vi "RemoteVI Logical Popups.vi"(0 "modal popups":T2(array[cluster]), 5 "d":cluster{"dx":i32, "dy":i32}) -> (4 "popups":T1)   [LabVIEW 2020, in "RemoteVI.lvlib"]
doc: "Builds the popups cluster that RemoteVI Service Client.vi and RemoteVI Post Input.vi work with: every window of modal popups at its LOGICAL position = real window position - d (the displacement by which the popups are currently moved, docs\\architecture.md, Popups), with its size, plus d itself. Pure."
uses:
  RemoteVI.lvlib
panel:
  in  "popups template":T1
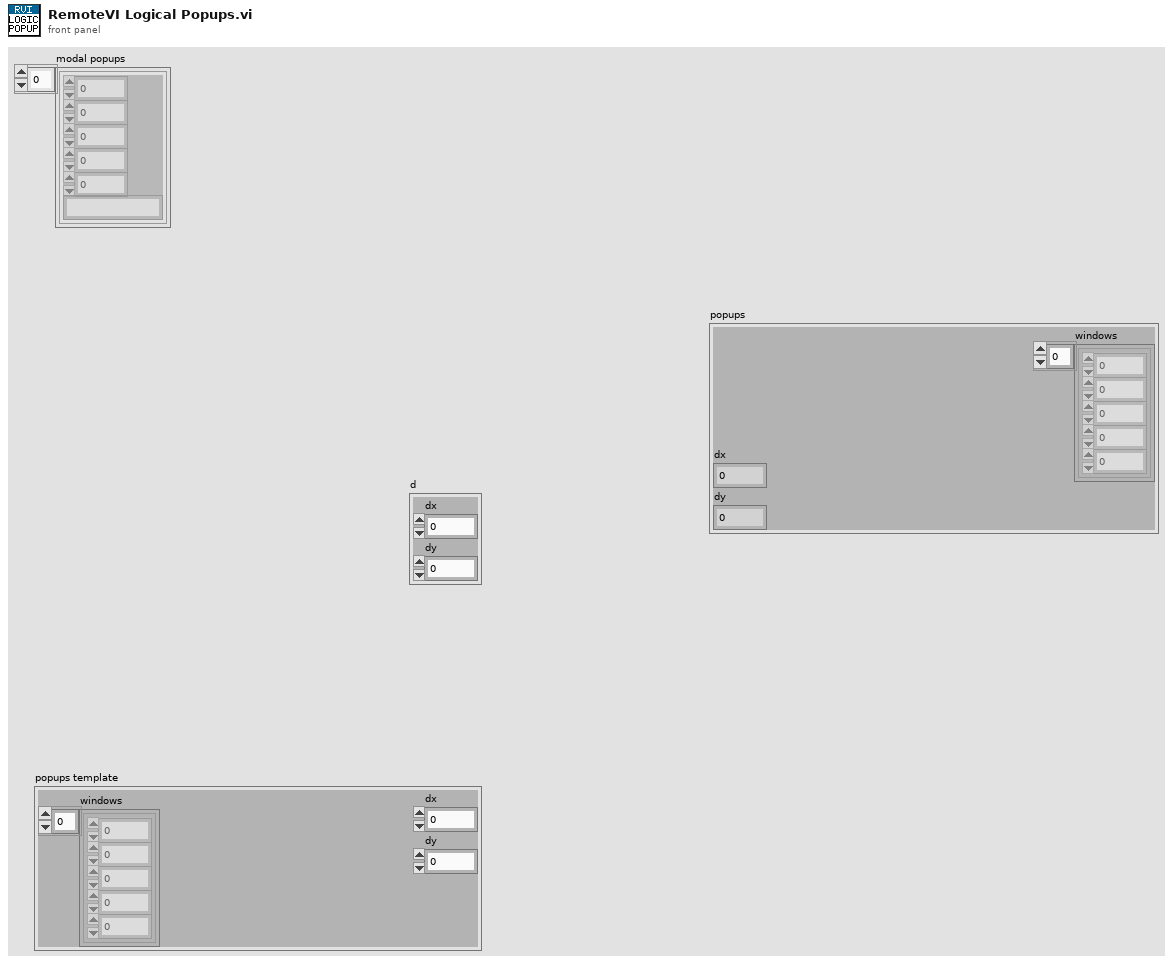
[diagram p1: front panel]
types:
  T1 = cluster{"windows":cluster{"hwnd":u64, "x":i32, "y":i32, "w":i32, "h":i32}[], "dx":i32, "dy":i32}
  T2 = cluster{"hwnd":u64, "x":i32, "y":i32, "w":i32, "h":i32, "class":string}[]
  T3 = cluster{"hwnd":u64, "x":i32, "y":i32, "w":i32, "h":i32}
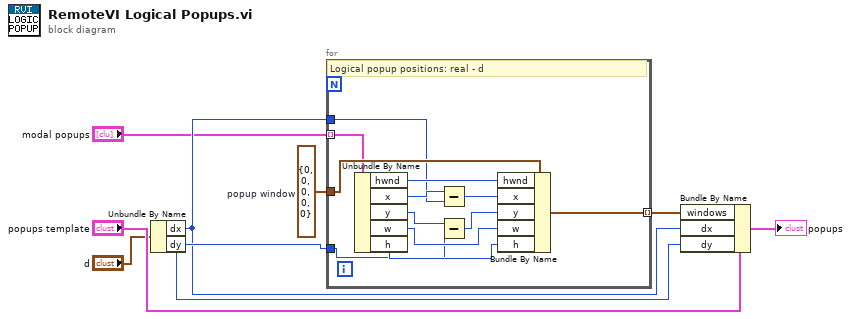
[diagram p0: block diagram]
diagram:
  w5 = T3 {"hwnd"=0, "x"=0, "y"=0, "w"=0, "h"=0}  # popup window
  n1 = Unbundle By Name("d") -> ("dx"=w3:i32, "dy"=w4:i32)
  n2 = for {
    tunnel: "modal popups" -> [w9] mode=indexing
    tunnel: w5 -> [w12]
    tunnel: w3 -> [w10]
    tunnel: w4 -> [w11]
    tunnel: [w20] -> w6 mode=indexing
    # "Logical popup positions: real - d"
    n3 = Unbundle By Name(w9) -> ("hwnd"=w13:u64, "x"=w14:i32, "y"=w15:i32, "w"=w16:i32, "h"=w17:i32)
    n4 = Subtract(x=w14, y=w10) -> (x-y=w18:i32)
    n5 = Subtract(x=w15, y=w11) -> (x-y=w19:i32)
    n6 = Bundle By Name(cluster=w12, "hwnd"=w13, "x"=w18, "y"=w19, "w"=w16, "h"=w17) -> (w20:T3)
  }
  n7 = Bundle By Name(cluster="popups template", "windows"=w6, "dx"=w3, "dy"=w4) -> (→"popups":T1)
